vi "CANsub_Set_Keepalive.vi"(8 "error in (no error)":errorcluster, 11 "fd":i32) -> (0 "error out":errorcluster, 3 "results":i32[](array[numeric]))   [LabVIEW 2021, in "CANsub_Common.lvlib"]
doc: "sets TCP keepalive on a socket before TLS: SO_KEEPALIVE on, first probe after 2 s idle, 1 s interval, 3 probes; TCP_USER_TIMEOUT 5 s. A dead peer is detected in about 5 s and the next TCP Read gives an error. 5005 if a setsockopt fails. Setup only.\n\nOn Windows the VI sets no option and returns an empty results array."
uses:
  CANsub_Common.lvlib
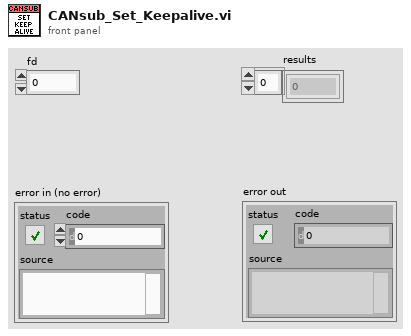
[diagram p1: front panel]
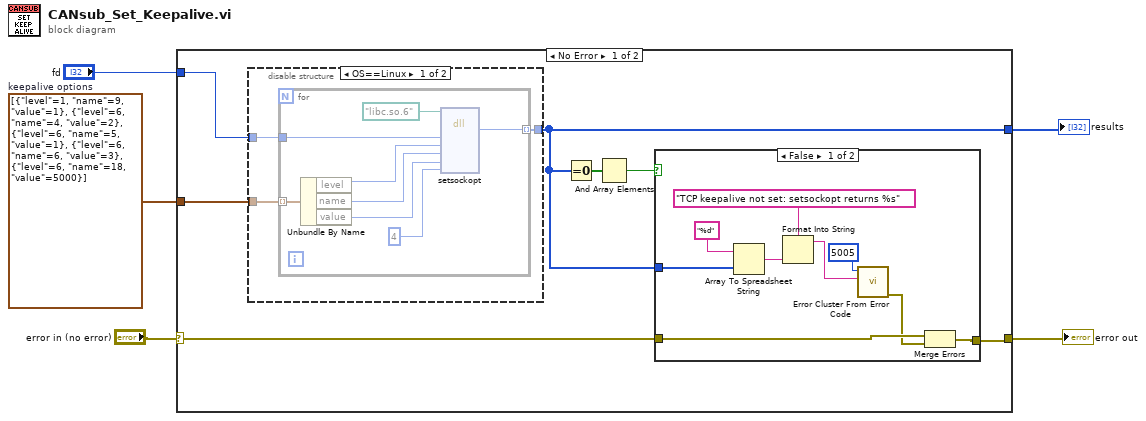
[diagram p0: block diagram]
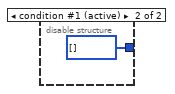
[diagram p2: hidden frame]
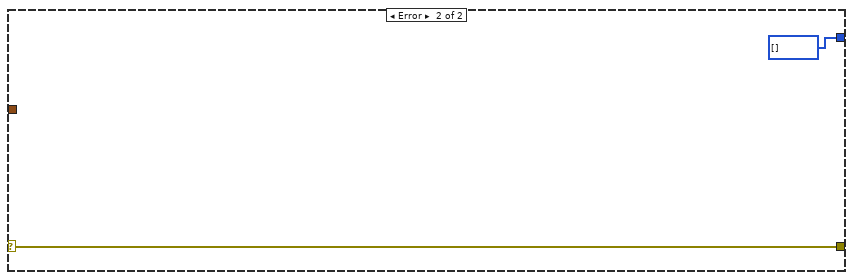
[diagram p4: hidden frame]
diagram:
  w2 = cluster{"level":i32, "name":i32, "value":i32}[] [{"level"=1, "name"=9, "value"=1}, {"level"=6, "name"=4, "value"=2}, {"level"=6, "name"=5, "value"=1}, {"level"=6, "name"=6, "value"=3}, {"level"=6, "name"=18, "value"=5000}]  # keepalive options
  n1 = case shown="No Error" "error in (no error)" {
    selector: "error in (no error)" -> [w7 w36]
    tunnel: [w8 w36] -> w4
    tunnel: [w6 i32[] [] ("results")] -> w3
    tunnel: w2 -> [w12 _]
    tunnel: "fd" -> [w11 _]
    frame No Error {
      n2 = disable-structure shown="OS==Linux" {
        disable-tunnel: w12 -> [w15 _]
        disable-tunnel: w11 -> [w14 _]
        disable-tunnel: [w13 i32[] []] -> w6
        frame condition #0 {
          n3 = for {
            tunnel: w15 -> [w23] mode=indexing
            tunnel: w14 -> [w22]
            tunnel: [w17] -> w13 mode=indexing
            n4 = Unbundle By Name(w23) -> ("level"=w21:i32, "name"=w20:i32, "value"=w19:i32)
            n5 = dll-call lib="libc.so.6" fn="setsockopt"(path in=path "libc.so.6", "sockfd"=w22, "level"=w21, "optname"=w20, "optval"=w19, "optlen"=u32 4) -> ("ret"=w17:i32)  [unwired: 7 in, 2 out]
          }
        }
        frame condition #1 (active) {
        }
      }
      n6 = Equal To 0?(x=w6) -> (x = 0?=w10:bool[])
      n7 = And Array Elements(Boolean array=w10) -> (logical AND=w9:bool)
      n8 = case shown="False" w9 {
        tunnel: [w28 w34] -> w8
        tunnel: w7 -> [w27 w34]
        tunnel: w6 -> [w32 _]
        frame False {
          n9 = Array To Spreadsheet String(array=w32, 3:"%d" ("delimiter (Tab)")) -> (spreadsheet string=w31:string)  [unwired: 1 in]
          n10 = Format Into String(format string="TCP keepalive not set: setsockopt returns %s", w31) -> (resulting string=w30:string)  [unwired: 2 in, 1 out]
          n11 = call <vilib>:"Error Cluster From Error Code.vi"("error message (\"\")"=w30, "error code (0)"=5005) -> ("error out"=w26:errorcluster)  [unwired: 7 in]
          n12 = Merge Errors(w27, w26) -> (w28:errorcluster)
        }
        frame True {
        }
      }
    }
    frame Error {
    }
  }
  "results" <- w3
  "error out" <- w4
